vi "Variable glob alertes pressions.vi"() -> ()   [LabVIEW 2022 SP3]
panel:
  out "Groupe ON":bool[](array[boolean])
  in  "groupes vide":T1(array[cluster]) {"valeur" format="%#_6e"}
  in  "Al vide en cours":bool
  out "Liste pres":string[](array[string])
  # "Alertes vide"
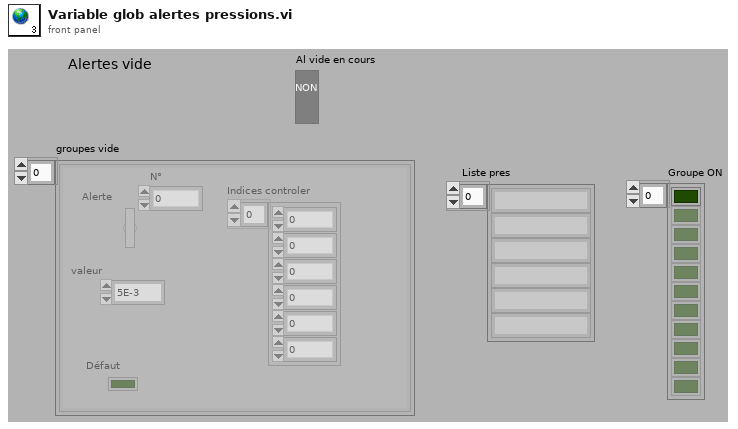
[diagram p1: front panel]
types:
  T1 = cluster{"Alerte":bool, "valeur ":dbl, "Défaut":bool, "Indices controler":i16[], "N°":u16}[]
diagram:
